vi "lvmcp_bind_array_elem.vi"() -> ()   [LabVIEW 2026]
doc: "Opens a VI through the active project's application instance, opens its front panel, replaces each named control (matched by Label.Text) with the given .ctl, saves the VI in place and restores the panel window state. Every error is wired."
panel:
  out "error out":errorcluster
  out "save vi error":errorcluster
  out "replace errors":errorcluster[](array[cluster])
  out "terminals bound":i32
  out "terminal names seen":string[](array[string])
  out "label errors":errorcluster[](array[cluster])
  out "open vi error":errorcluster
  in  "error in":errorcluster
  in  "ctl paths":string
  in  "terminal names":string
  in  "vi path":string
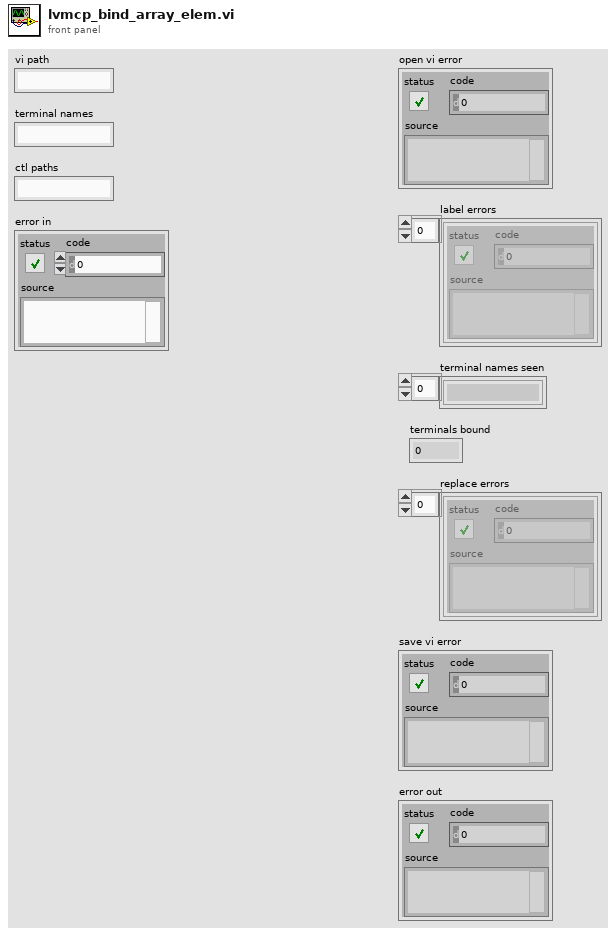
[diagram p1: front panel]
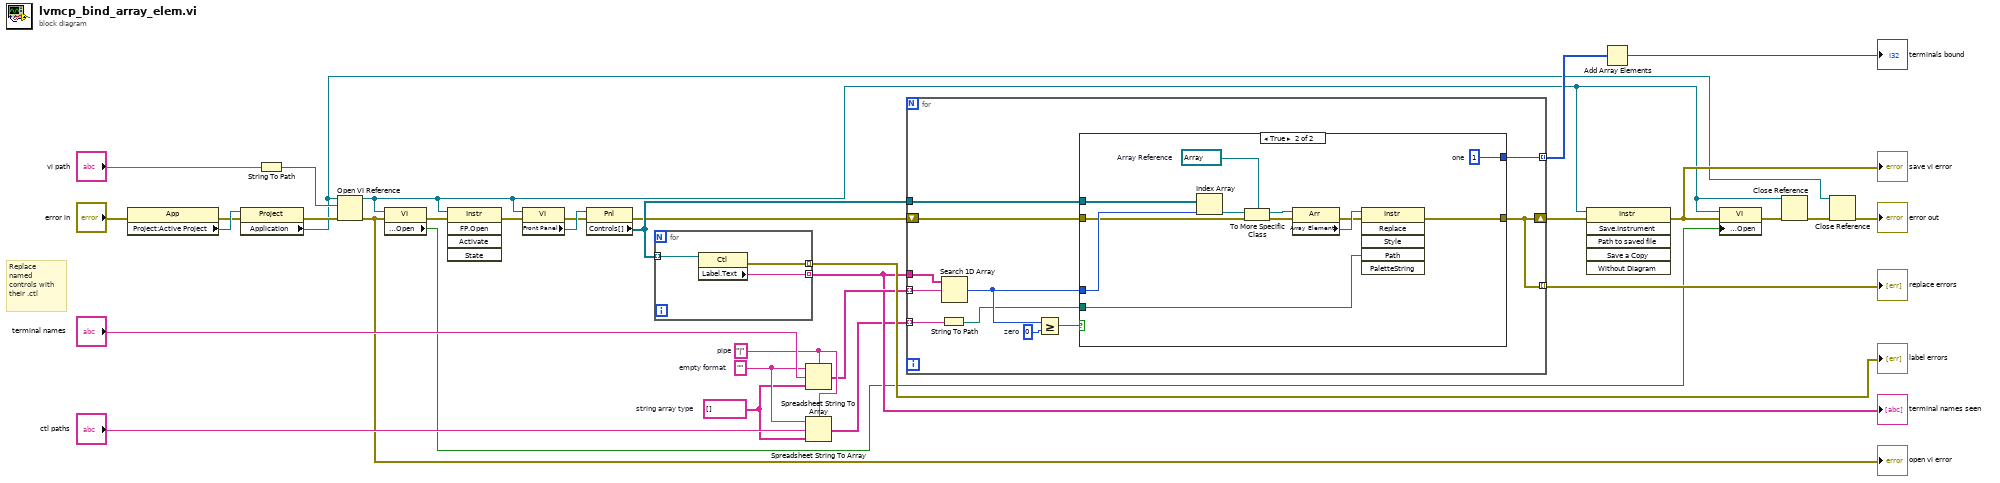
[diagram p0: block diagram]
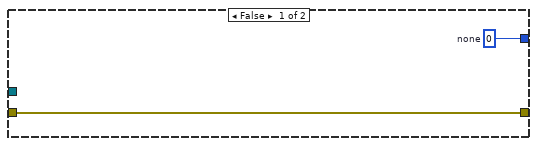
[diagram p2: hidden frame]
diagram:
  w27 = string[] []  # string array type
  w26 = "|"  # pipe
  w29 = ""  # empty format
  # "Replace named controls with their .ctl"
  n1 = property class="App"(error in="error in") -> (error out=w31:errorcluster, "Project:Active Project"=w32:refnum<vi>)  [unwired: 1 in, 1 out]
  n2 = property class="Project"(reference=w32, error in=w31) -> (error out=w23:errorcluster, "Application"=w3:refnum<vi>)  [unwired: 1 out]
  n3 = String To Path(string="vi path") -> (path=w24:path)
  n4 = Open VI Reference(application reference (local)=w3, vi path=w24, error in (no error)=w23) -> (vi reference=w5:refnum<vi>, error out=w22:errorcluster)  [unwired: 3 in]
  "open vi error" <- w22
  n5 = property class="VI"(reference=w5, error in=w22) -> (error out=w21:errorcluster, "Front Panel Window:Open"=w6:bool)  [unwired: 1 out]
  n6 = invoke class="Instr" method="FP.Open"(reference=w5, error in=w21) -> (error out=w20:errorcluster)  [unwired: 3 in, 4 out]
  n7 = property class="VI"(reference=w5, error in=w20) -> (error out=w18:errorcluster, "Front Panel"=w19:refnum<vi>)  [unwired: 1 out]
  n8 = property class="Pnl"(reference=w19, error in=w18) -> (error out=w12:errorcluster, "Controls[]"=w14:refnum<vi>[])  [unwired: 1 out]
  n9 = for {
    tunnel: w14 -> [w36] mode=indexing
    tunnel: [w35] -> w15 mode=indexing
    tunnel: [w34] -> w17 mode=indexing
    n10 = property class="Ctl"(reference=w36) -> (error out=w34:errorcluster, "Label.Text"=w35:string)  [unwired: 1 in, 1 out]
  }
  "label errors" <- w17
  "terminal names seen" <- w15
  n11 = Spreadsheet String To Array(delimiter (Tab)=w26, format string=w29, spreadsheet string="terminal names", array type (2D Dbl)=w27) -> (array=w16:string[])
  n12 = Spreadsheet String To Array(delimiter (Tab)=w26, format string=w29, spreadsheet string="ctl paths", array type (2D Dbl)=w27) -> (array=w13:string[])
  n13 = for {
    tunnel: w16 -> [w45] mode=indexing
    tunnel: w15 -> [w46]
    tunnel: w14 -> [w43]
    tunnel: w13 -> [w47] mode=indexing
    shift-right: [w37] -> w8
    shift-left: w12 -> [w40]
    tunnel: [w38] -> w11 mode=indexing
    tunnel: [w37] -> w9 mode=indexing
    w44 = 0  # zero
    n14 = String To Path(string=w47) -> (path=w41:path)
    n15 = Search 1D Array(1D array=w46, element=w45) -> (index of element=w42:i32)  [unwired: 1 in]
    n16 = Greater Or Equal?(x=w42, y=w44) -> (x >= y?=w39:bool)
    n17 = case shown="True" w39 {
      tunnel: w43 -> [_ w61]
      tunnel: w42 -> [_ w60]
      tunnel: w41 -> [_ w52]
      tunnel: w40 -> [w48 w58]
      tunnel: [w49 w51] -> w38
      tunnel: [w48 w50] -> w37
      frame False {
        w49 = 0  # none
      }
      frame True {
        w51 = 1  # one
        w57 = refnum<vi> refnum  # Array Reference
        n18 = Index Array(array=w61, index=w60) -> (element=w59:refnum<vi>)
        n19 = To More Specific Class(target class=w57, reference=w59, error in=w58) -> (specific class reference=w56:refnum<vi>, error out=w55:errorcluster)
        n20 = property class="Arr"(reference=w56, error in=w55) -> (error out=w53:errorcluster, "Array Element"=w54:refnum<vi>)  [unwired: 1 out]
        n21 = invoke class="Instr" method="Replace"(reference=w54, error in=w53, "Path"=w52) -> (error out=w50:errorcluster)  [unwired: 3 in, 5 out]
      }
    }
  }
  "replace errors" <- w9
  n22 = invoke class="Instr" method="Save.Instrument"(reference=w5, error in=w8) -> (error out=w7:errorcluster)  [unwired: 4 in, 5 out]
  "save vi error" <- w7
  n23 = Add Array Elements(numeric array=w11) -> (sum=→"terminals bound":i32)
  n24 = property class="VI"(reference=w5, error in=w7, "Front Panel Window:Open"=w6) -> (error out=w4:errorcluster)  [unwired: 1 out]
  n25 = Close Reference(reference=w5, error in (no error)=w4) -> (error out=w2:errorcluster)
  n26 = Close Reference(reference=w3, error in (no error)=w2) -> (error out=→"error out":errorcluster)
